vi "D_Close.vi"(8 "error in (no error)":errorcluster, 11 "bIDList":u8[](array[numeric])) -> (0 "error out":errorcluster, 4 "TorF":i32)   [LabVIEW 2018]
uses:
  hpkSLMdaLV.dll
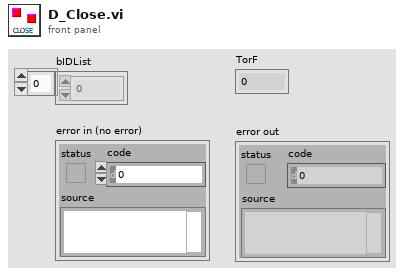
[diagram p1: front panel]
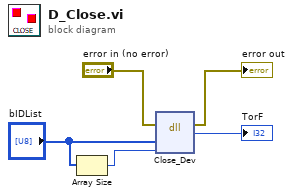
[diagram p0: block diagram]
diagram:
  n1 = Array Size(array="bIDList") -> (size(s)=w2:i32)
  n2 = dll-call lib="PTH2ﾅunc \\\\K45292-FS\\Data\n荳ｭ遐猫COSpost譛晉ｨｲ\n08_LabVIEW!00_繝ｩ繝懊ン繝･繝ｼ繝励Ο繧ｰ繝ｩ繝LabVIEW2018 LCOS_DriverV3.0_Hardware_ControlUSB_Multi-ControlHardwareControl_LVhpkSLMdaLV.dll" fn="Close_Dev"(error in="error in (no error)", "bIDList"="bIDList", "bIDSize"=w2) -> (error out=→"error out":errorcluster, "返り値タイプ"=→"TorF":i32)  [unwired: 4 in, 1 out]
